vi "Set Representation.vi"(8 "error in":errorcluster, 11 "Numeric in":refnum<class "Numeric.lvclass">) -> (0 "error out":errorcluster, 3 "Numeric out":refnum<class "Numeric.lvclass">)   [LabVIEW 2026, in "Numeric.lvclass"]
doc: "Set representation of numeric element."
uses:
  Numeric.lvclass
  <vilib>/numeric/LVNumericRepresentation.ctl
  Numeric.lvclass/Numeric.ctl
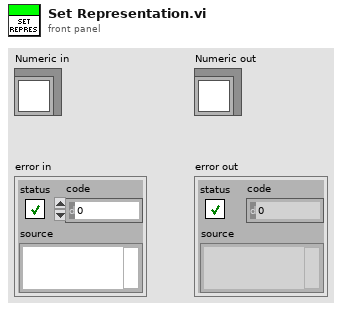
[diagram p1: front panel]
types:
  T1 = typedef "LVNumericRepresentation.ctl" = enum32{"Extended Precision", "Double Precision", "Single Precision", "Long", "Word", "Byte", "Unsigned Long", "Unsigned Word", "Unsigned Byte", "Complex Extended", "Complex Double", "Complex Single", "Quad", "Unsigned Quad", "Fixed-Point"}
  T2 = typedef "Data types--enum.ctl" = enum16{"int", "float", "bool", "str", "TypedDict", "np.bool_", "np.int8", "np.int16", "np.int32", "np.int64", "np.uint8", "np.uint16", "np.uint32", "np.uint64", "np.float32", "np.float64", "np.str_"}
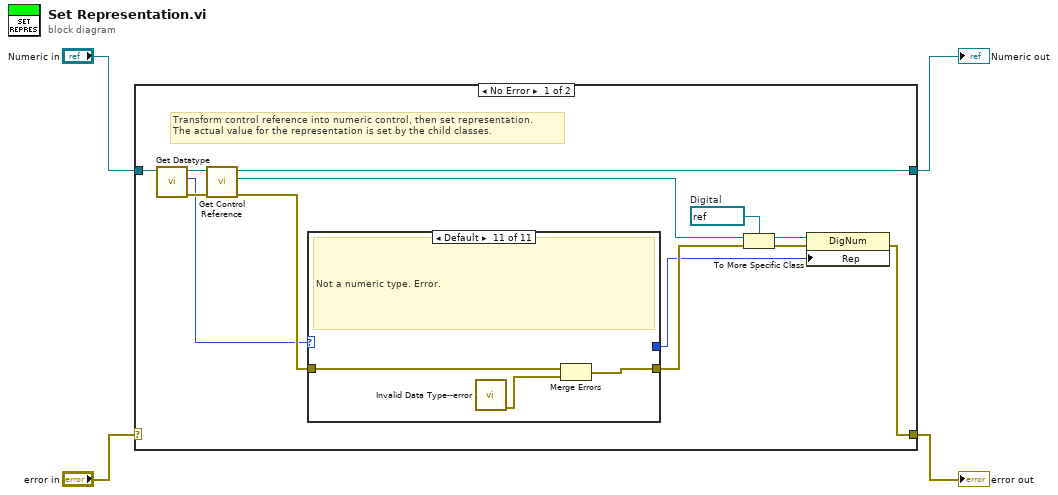
[diagram p0: block diagram]
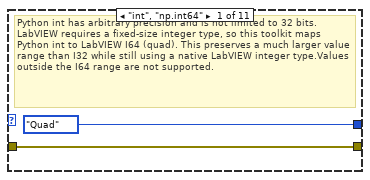
[diagram p2: hidden frame]
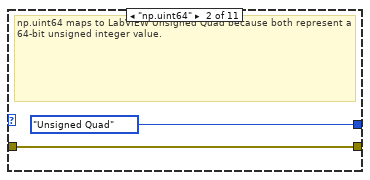
[diagram p3: hidden frame]
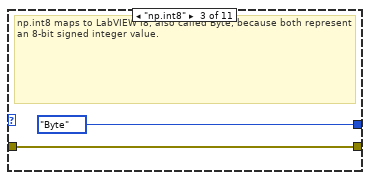
[diagram p4: hidden frame]
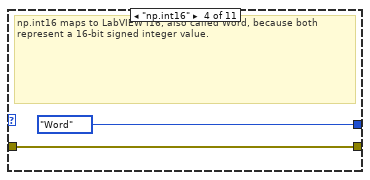
[diagram p5: hidden frame]
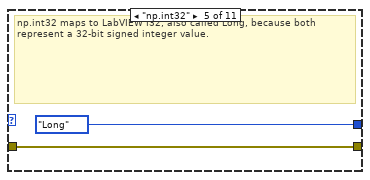
[diagram p6: hidden frame]
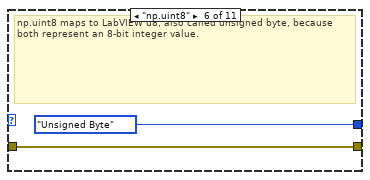
[diagram p7: hidden frame]
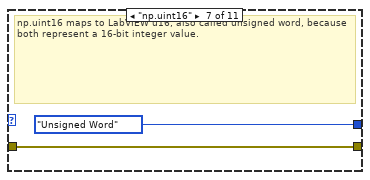
[diagram p8: hidden frame]
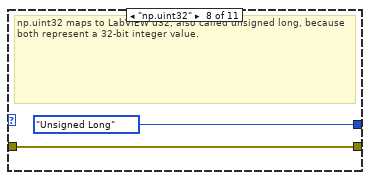
[diagram p9: hidden frame]
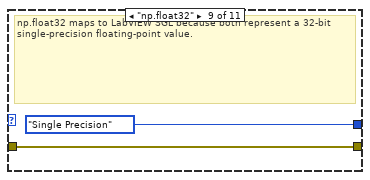
[diagram p10: hidden frame]
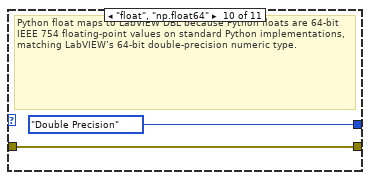
[diagram p11: hidden frame]
diagram:
  n1 = case shown="No Error" "error in" {
    selector: "error in" -> [_ w42]
    tunnel: [w16 w42] -> w3
    tunnel: [w6 w41] -> w1
    tunnel: "Numeric in" -> [w9 w41]
    frame No Error {
      w12 = refnum<vi> refnum  # Digital
      # "Transform control reference into numeric control, then set representation.\nThe actual value for the representation is set by the child classes."
      n2 = call-dynamic "Get Datatype.vi"("Element in"=w9) -> ("error out"=w14:errorcluster, "Datatype"=w8:T2, "Element out"=w7:refnum<class "Numeric.lvclass">)  [unwired: 8 in]
      n3 = call-dynamic "Get Control Reference.vi"("error in"=w14, "Element in"=w7) -> ("error out"=w13:errorcluster, "Control Reference"=w5:refnum<vi>, "Element out"=w6:refnum<class "Numeric.lvclass">)  [unwired: 7 in]
      n4 = case shown="Default" w8 {
        tunnel: [LVNumericRepresentation."Quad" ("Representation") LVNumericRepresentation."Unsigned Quad" ("Representation") LVNumericRepresentation."Byte" ("Representation") LVNumericRepresentation."Word" ("Representation") LVNumericRepresentation."Long" ("Representation") LVNumericRepresentation."Unsigned Byte" ("Representation") LVNumericRepresentation."Unsigned Word" ("Representation") LVNumericRepresentation."Unsigned Long" ("Representation") LVNumericRepresentation."Single Precision" ("Representation") LVNumericRepresentation."Double Precision" ("Representation") _] -> w10
        tunnel: w13 -> [w19 w21 w23 w25 w27 w29 w31 w33 w35 w37 w40]
        tunnel: [w19 w21 w23 w25 w27 w29 w31 w33 w35 w37 w38] -> w15
        frame "int", "np.int64" {
          # "Python int has arbitrary precision and is not limited to 32 bits. LabVIEW requires a fixed-size integer type, so this toolkit maps Python int to LabVIEW I64 (quad). This preserves a much larger value range than I32 while still using a native LabVIEW integer type.Values outside the I64 range are not supported."
        }
        frame "np.uint64" {
          # "np.uint64 maps to LabVIEW Unsigned Quad because both represent a 64-bit unsigned integer value."
        }
        frame "np.int8" {
          # "np.int8 maps to LabVIEW I8, also called Byte, because both represent an 8-bit signed integer value."
        }
        frame "np.int16" {
          # "np.int16 maps to LabVIEW I16, also called Word, because both represent a 16-bit signed integer value."
        }
        frame "np.int32" {
          # "np.int32 maps to LabVIEW I32, also called Long, because both represent a 32-bit signed integer value."
        }
        frame "np.uint8" {
          # "np.uint8 maps to LabVIEW u8, also called unsigned byte, because both represent an 8-bit integer value."
        }
        frame "np.uint16" {
          # "np.uint16 maps to LabVIEW u16, also called unsigned word, because both represent a 16-bit integer value."
        }
        frame "np.uint32" {
          # "np.uint32 maps to LabVIEW u32, also called unsigned long, because both represent a 32-bit integer value."
        }
        frame "np.float32" {
          # "np.float32 maps to LabVIEW SGL because both represent a 32-bit single-precision floating-point value."
        }
        frame "float", "np.float64" {
          # "Python float maps to LabVIEW DBL because Python floats are 64-bit IEEE 754 floating-point values on standard Python implementations, matching LabVIEW’s 64-bit double-precision numeric type."
        }
        frame Default {
          # "Not a numeric type. Error."
          n5 = call "Invalid Data Type--error.vi"() -> ("error out"=w39:errorcluster)  [unwired: 11 in]
          n6 = Merge Errors(w40, w39) -> (w38:errorcluster)
        }
      }
      n7 = To More Specific Class(target class=w12, reference=w5, error in=w15) -> (specific class reference=w11:refnum<vi>, error out=w17:errorcluster)
      n8 = property on="Property Node" class="DigNum"(reference=w11, error in=w17, "Rep"=w10) -> (error out=w16:errorcluster)  [unwired: 1 out]
    }
    frame Error {
    }
  }
  "error out" <- w3
  "Numeric out" <- w1
